vi "Write Results CSV.vi"(5 "overall verdict":string, 7 "Step Results":T1[](array[typedef]), 8 "error in":errorcluster, 9 "rig_id":string, 10 "sequence_id":string, 11 "results folder":path) -> (0 "error out":errorcluster, 3 "file path":path)   [LabVIEW 2026]
doc: "Writes the step results as a CSV report to results folder named sequence_id_YYYYMMDD_HHMMSS.csv, creating the folder if needed (an existing folder is not an error). Content: a header row step_no,step_name,result,reason,measured,target,duration_ms, a rig_id line, one row per Step Result and a final line OVERALL with the verdict. An empty folder path returns error 7 and writes nothing; an incoming error skips the write. AF-free."
uses:
  Typedefs/Step Result.ctl
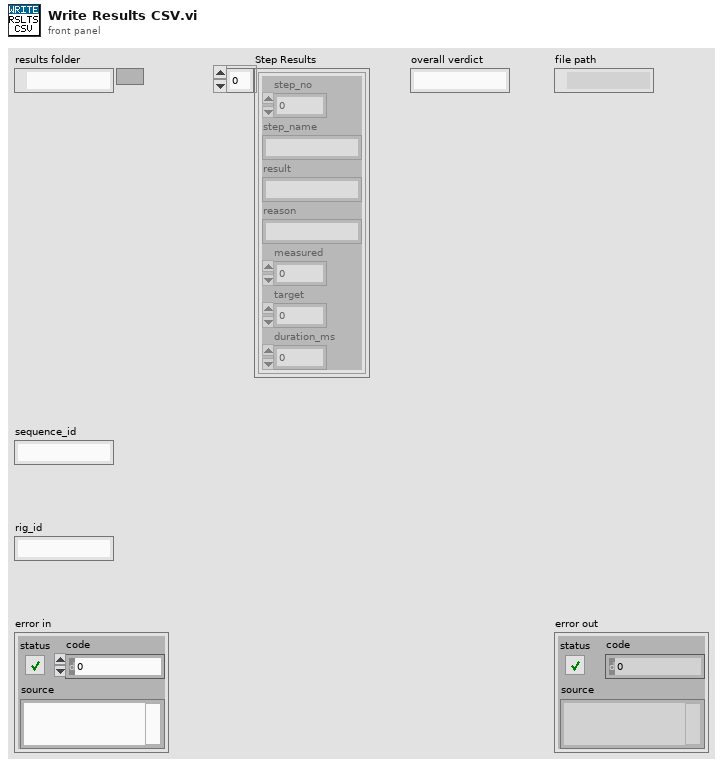
[diagram p1: front panel]
types:
  T1 = typedef "Step Result.ctl" = cluster{"step_no":i32, "step_name":string, "result":string, "reason":string, "measured":dbl, "target":dbl, "duration_ms":dbl}
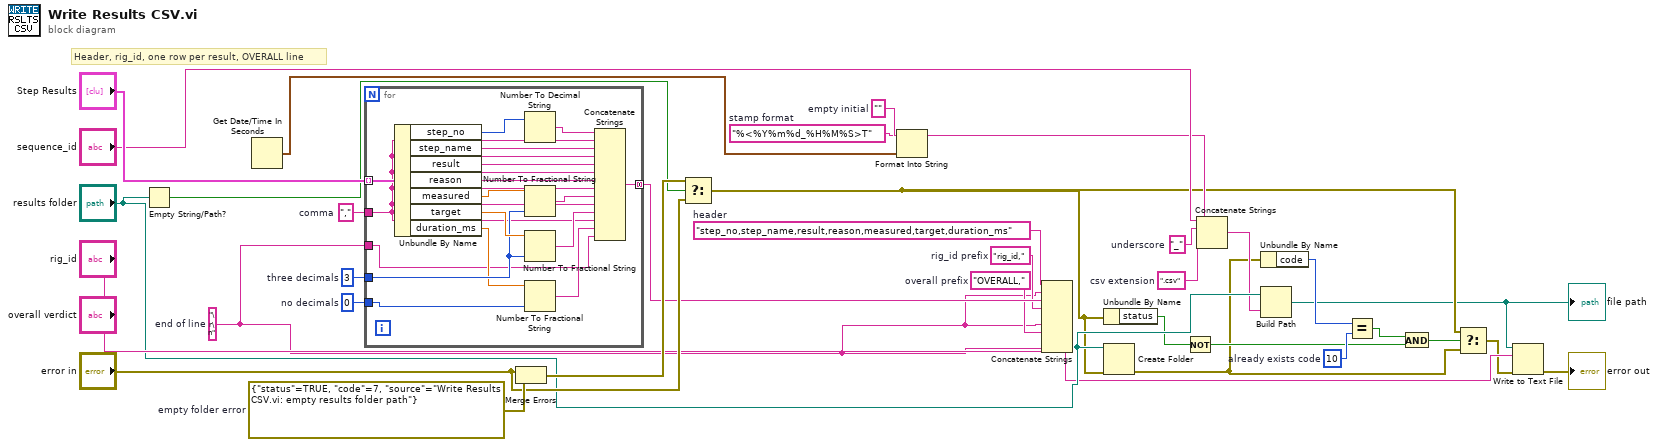
[diagram p0: block diagram]
diagram:
  w21 = "OVERALL,"  # overall prefix
  w23 = "rig_id,"  # rig_id prefix
  w25 = "step_no,step_name,result,reason,measured,target,duration_ms"  # header
  w32 = 0  # no decimals
  w33 = 3  # three decimals
  w19 = "\r\n"  # end of line
  w34 = ","  # comma
  w15 = ".csv"  # csv extension
  w17 = "_"  # underscore
  w31 = ""  # empty initial
  w29 = "%<%Y%m%d_%H%M%S>T"  # stamp format
  w10 = 10  # already exists code
  w36 = errorcluster {"status"=TRUE, "code"=7, "source"="Write Results CSV.vi: empty results folder path"}  # empty folder error
  # "Header, rig_id, one row per result, OVERALL line"
  n1 = Empty String/Path?(string/path="results folder") -> (empty?=w27:bool)
  n2 = Get Date/Time In Seconds() -> (seconds since 1Jan1904=w30:timestamp)
  n3 = for {
    tunnel: "Step Results" -> [w53] mode=indexing
    tunnel: w34 -> [w40]
    tunnel: w19 -> [w38]
    tunnel: w33 -> [w49]
    tunnel: w32 -> [w47]
    tunnel: [w37] -> w24 mode=concatenating
    n4 = Unbundle By Name(w53) -> ("step_no"=w52:i32, "step_name"=w45:string, "result"=w44:string, "reason"=w43:string, "measured"=w51:dbl, "target"=w50:dbl, "duration_ms"=w48:dbl)
    n5 = Number To Decimal String(number=w52) -> (decimal integer string=w46:string)  [unwired: 1 in]
    n6 = Number To Fractional String(number=w51, precision (6)=w49) -> (F-format string=w42:string)  [unwired: 2 in]
    n7 = Number To Fractional String(number=w50, precision (6)=w49) -> (F-format string=w41:string)  [unwired: 2 in]
    n8 = Number To Fractional String(number=w48, precision (6)=w47) -> (F-format string=w39:string)  [unwired: 2 in]
    n9 = Concatenate Strings(w46, w40, w45, w40, w44, w40, w43, w40, w42, w40, w41, w40, w39, w38) -> (w37:string)
  }
  n10 = Merge Errors("error in", w36) -> (w28:errorcluster)
  n11 = Select(t=w28, s=w27, f="error in") -> (s? t:f=w7:errorcluster)
  n12 = Format Into String(format string=w29, initial string=w31, w30) -> (resulting string=w16:string)  [unwired: 1 in, 1 out]
  n13 = Concatenate Strings(w25, w19, w24, w23, "rig_id", w19, w21, "overall verdict", w19) -> (w4:string)
  n14 = Unbundle By Name(w7) -> ("status"=w12:bool)
  n15 = Create Folder(path (use dialog)="results folder", error in=w7) -> (error out=w5:errorcluster)  [unwired: 1 in, 2 out]
  n16 = Not(x=w12) -> (.not. x?=w8:bool)
  n17 = Concatenate Strings("sequence_id", w17, w16, w15) -> (w13:string)
  n18 = Unbundle By Name(w5) -> ("code"=w11:i32)
  n19 = Build Path(base path="results folder", name or relative path=w13) -> (appended path=w2:path)
  "file path" <- w2
  n20 = Equal?(x=w11, y=w10) -> (x = y?=w9:bool)
  n21 = And(x=w9, y=w8) -> (x .and. y?=w6:bool)
  n22 = Select(t=w7, s=w6, f=w5) -> (s? t:f=w3:errorcluster)
  n23 = Write to Text File(file (use dialog)=w2, text=w4, error in=w3) -> (error out=→"error out":errorcluster)  [unwired: 1 in, 2 out]
